vi "csb ws state init.vi"(8 "error in (no error)":errorcluster, 10 "state_size":i32, 11 "state":u8[](array[numeric])) -> (0 "error out":errorcluster, 2 "function return":i32, 3 "state_out":u8[](array[numeric]))   [LabVIEW 2021, in "CANsub_Codec.lvlib"]
doc: "int32_t csb_ws_state_init(uint8_t *state, int32_t state_size);"
uses:
  CANsub_Codec.lvlib
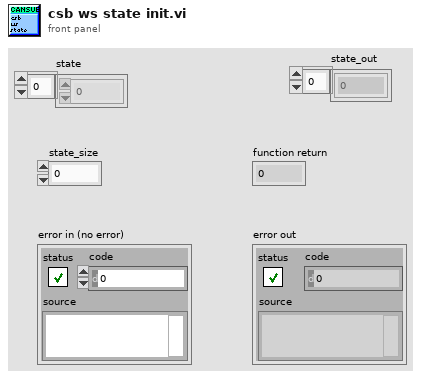
[diagram p1: front panel]
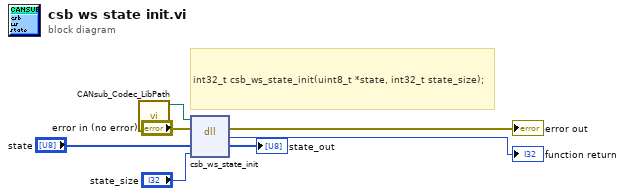
[diagram p0: block diagram]
diagram:
  # "int32_t csb_ws_state_init(uint8_t *state, int32_t state_size);"
  n1 = call "CANsub_Codec_LibPath.vi"() -> ("Path"=w1:path)  [unwired: 11 in]
  n2 = dll-call lib="libcansub_codec.*" fn="csb_ws_state_init"(path in=w1, error in="error in (no error)", "state"="state", "state_size"="state_size") -> (error out=→"error out":errorcluster, "return type"=→"function return":i32, "state"=→"state_out":u8[])  [unwired: 2 in, 1 out]
